vi "write bool temp.vi"(9 "data":variant, 10 "station":string, 11 "URL":string) -> (2 "Value":u8[](array[numeric]), 3 "ok?":bool)   [LabVIEW 2012]
uses:
  read_Array.vi
  write_Array.vi
  Globals/Global.vi
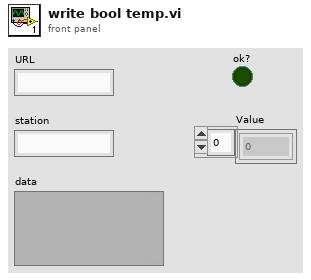
[diagram p1: front panel]
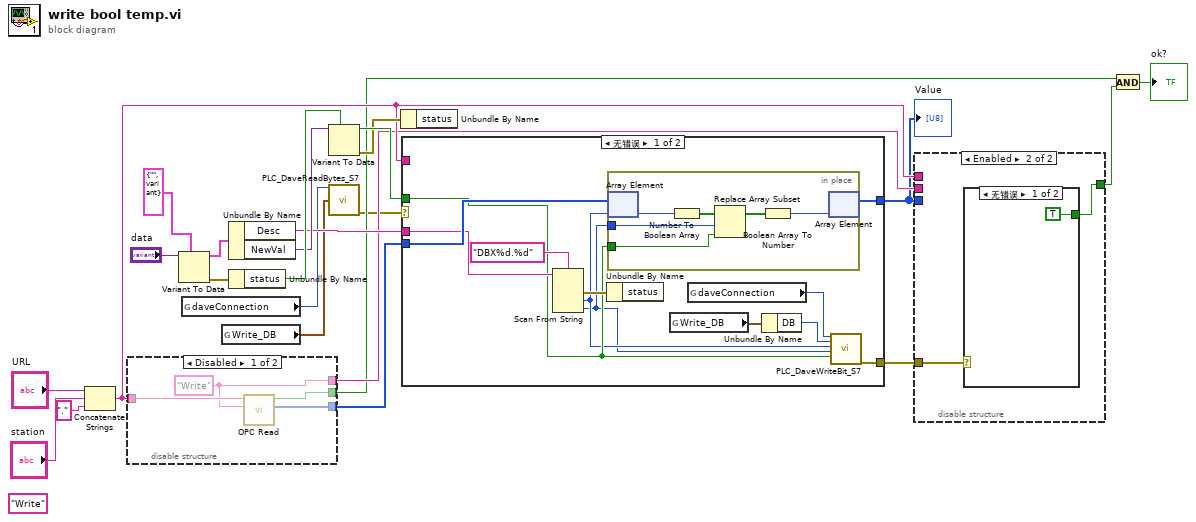
[diagram p0: block diagram]
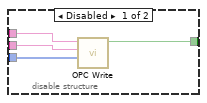
[diagram p3: hidden frame]
diagram:
  (unwired) "Write" ("Address")
  n1 = Concatenate Strings("URL", "station", "." ("string")) -> (w10:string)
  n2 = disable-structure shown="Disabled" {
    disable-tunnel: [w27 _] -> w13
    disable-tunnel: w10 -> [w26 _]
    disable-tunnel: [w25 _] -> w9
    disable-tunnel: [w24 _] -> w7
    frame Disabled {
      w25 = "Write" ("Address")
      n3 = call-poly "OPC Read.vi"("Address"=w25, "URL"=w26) -> ("Value"=w27:u8[], "ok?"=w24:bool)  [unwired: 7 in, 1 out]
    }
    frame Enabled {
    }
  }
  n4 = Variant To Data(type=cluster{"Desc":string, "NewVal":variant} {"Desc"="", "NewVal"=variant} ("output cluster"), Variant="data") -> (data=w17:cluster{"Desc":string, "NewVal":variant}, error out=w15:errorcluster)  [unwired: 1 in]
  n5 = global read "Global.vi" "daveConnection"() -> (w3:i64)
  n6 = global read "Global.vi" "Write_DB"() -> (w4:cluster{"DB":i32, "start":i32, "len":i32})
  n7 = Unbundle By Name(w17) -> ("Desc"=w18:string, "NewVal"=w19:variant)
  n8 = Unbundle By Name(w15) -> ("status"=w20:bool)
  n9 = Variant To Data(type=w20, Variant=w19) -> (data=w22:bool, error out=w21:errorcluster)  [unwired: 1 in]
  n10 = call "PLC_DaveReadBytes_S7.vi"("daveConnection in"=w3, "地址"=w4) -> ("error out"=w2:errorcluster)  [unwired: 10 in, 3 out]
  n11 = Unbundle By Name(w21) -> ()  [unwired: 1 out]
  n12 = case shown="无错误" w2 {
    selector: w2 -> [_ w46]
    tunnel: w10 -> [_ _]
    tunnel: w13 -> [w39 _]
    tunnel: w22 -> [w31 _]
    tunnel: w18 -> [w37 _]
    tunnel: [w35 _] -> w8
    tunnel: [w30 w46] -> w1
    frame No Error {
      n13 = Scan From String(format string="DBX%d.%d" ("regular expression"), input string=w37) -> (error out=w36:errorcluster, output 1=w29:i32, output 2=w28:i32)  [unwired: 4 in, 2 out]
      n14 = Unbundle By Name(w36) -> ()  [unwired: 1 out]
      n15 = in-place {
        in-place-border: w28 -> [w43]
        in-place-border: w31 -> [w42]
        n16 = in-place-array #1(w39, w29) -> (w45:u8)
        n17 = Number To Boolean Array(number=w45) -> (Boolean array=w44:bool[])
        n18 = Replace Array Subset(array=w44, new element=w42, index=w43) -> (w41:bool[])
        n19 = Boolean Array To Number(Boolean array=w41) -> (number=w40:u32)
        n20 = in-place-array #1(w40) -> (w35:u8[])  [unwired: 1 out]
      }
      n21 = global read "Global.vi" "Write_DB"() -> (w32:cluster{"DB":i32, "start":i32, "len":i32})
      n22 = global read "Global.vi" "daveConnection"() -> (w33:i64)
      n23 = Unbundle By Name(w32) -> ("DB"=w34:i32)
      n24 = call "PLC_DaveWriteBit_S7.vi"("daveConnection IN"=w33, "DB"=w34, "byte"=w29, "bit"=w28, "value"=w31) -> ("error out"=w30:errorcluster)  [unwired: 12 in, 2 out]
    }
    frame Error {
    }
  }
  "Value" <- w8
  n25 = disable-structure shown="Enabled" {
    disable-tunnel: w10 -> [w50 _]
    disable-tunnel: w9 -> [w49 _]
    disable-tunnel: [w48 w52] -> w6
    disable-tunnel: w8 -> [w47 _]
    disable-tunnel: w1 -> [_ w51]
    frame Disabled {
      n26 = call-poly "OPC Write.vi"("Value"=w47, "Address"=w49, "URL"=w50) -> ("ok?"=w48:bool)  [unwired: 7 in, 1 out]
    }
    frame Enabled {
      n27 = case shown="无错误" w51 {
        tunnel: [TRUE ("ok?") _] -> w52
        frame No Error {
        }
        frame Error {
        }
      }
    }
  }
  n28 = And(x=w7, y=w6) -> (x .and. y?=→"ok?":bool)
